vi "Main.vi"() -> ()   [LabVIEW 2020]
doc: "Example application with authentication."
uses:
  Type Definitions/States--enum.ctl
  Type Definitions/Loop Data--cluster.ctl
  <vilib>/gRPC/LabVIEW gRPC Library/Shared/grpcId.ctl
  <vilib>/sklein/WebView2/Webview2 Lib/WebView2 Control Object/WebView2 Control.lvclass
  <vilib>/Utility/miscctls.llb/LVPointTypeDef.ctl
  <vilib>/Utility/miscctls.llb/LVRectTypeDef.ctl
  grpc-auth_client/RPC Messages/auth_SubscribeLoginRequest.ctl
  grpc-auth_client/RPC Messages/auth_ValidateTokenRequest.ctl
  grpc-auth_client/RPC Messages/auth_RefreshTokenRequest.ctl
  grpc-auth_client/RPC Messages/auth_LogoutRequest.ctl
  e78014cf-5a62-4ef9-a1df-b3f489fcdea7.vi
  32d3baa6-2010-401a-92df-034dbfa07a08.vi
  <vilib>/Comparison/Equal/Equal Functor/Equal Functor.lvclass
  grpc-auth_client/grpc-auth_client.lvlib
  <vilib>/gRPC/LabVIEW gRPC Library/grpc-lvsupport-release.lvlib
  C:/Program Files (x86)/National Instruments/LabVIEW 2020/vi.lib/sklein/WebView2/Libs/Microsoft.Web.WebView2.WinForms.dll
  Program Files (x86)/National Instruments/LabVIEW 2020/vi.lib/sklein/WebView2/Libs/Microsoft.Web.WebView2.WinForms.dll
panel:
  in  "Tab Control":enum32{"Login", "Run"}(tab)
  in  "WebView2":refnum<k24>(container)
  in  "Extend":bool
  out "Access Expires At":string
  out "Current User":string
  out "In Operation":bool
  in  "operate":bool
  in  "debug":bool
  out "Debugging":bool
  in  "logout":bool
  # "Operation is only allowed\nfor members of group\n\"Operator\""
  # "Debugging is only allowed\nfor members of group\n\"Developers\""
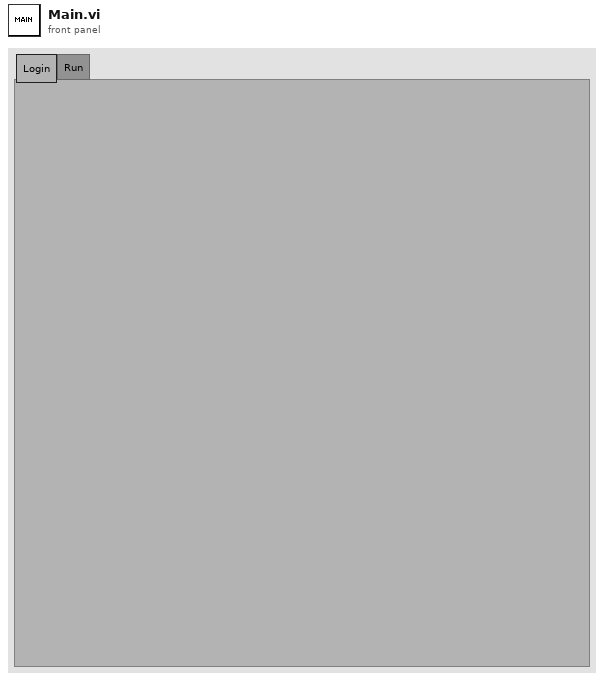
[diagram p1: front panel]
types:
  T1 = typedef "Loop Data--cluster.ctl" = cluster{"gRPC ID":T2, "Login Session ID":string, "Access Token":string, "Login Call ID":T2, "WebView2 Control":refnum<class "WebView2 Control.lvclass">}
  T2 = typedef "grpc-lvsupport-release.lvlib/grpcId.ctl" = u64
  T3 = typedef "States--enum.ctl" = enum16{"Init", "Login", "Idle", "Error", "Exit", "Begin SubscribeLogin", "End SubscribeLogin", "Logout"}
  T4 = typedef "LVRectTypeDef.ctl" = cluster{"Left":i16, "Top":i16, "Right":i16, "Bottom":i16}
  T5 = typedef "LVPointTypeDef.ctl" = cluster{"Horizontal":i16, "Vertical":i16}
  T6 = typedef "grpc-auth_client.lvlib/auth_SubscribeLoginRequest.ctl" = cluster{"session_id":string}
  T7 = typedef "grpc-auth_client.lvlib/auth_ValidateTokenRequest.ctl" = cluster{"access_token":string}
  T8 = typedef "grpc-auth_client.lvlib/auth_RefreshTokenRequest.ctl" = cluster{"access_token":string}
  T9 = typedef "grpc-auth_client.lvlib/auth_LogoutRequest.ctl" = cluster{"access_token":string}
  T10 = typedef "grpc-auth_client.lvlib/auth_StartLoginResponse.ctl" = cluster{"ok":bool, "error":string, "session_id":string, "login_url":string, "expires_at":i64}
  T11 = typedef "grpc-auth_client.lvlib/auth_ValidateTokenResponse.ctl" = cluster{"valid":bool, "error":string, "user_id":string, "groups":string[]}
  T12 = typedef "grpc-auth_client.lvlib/auth_SubscribeLoginResponse.ctl" = cluster{"ok":bool, "error":string, "status":T13, "access_token":string, "access_expires_at":i64, "username":string}
  T13 = typedef "grpc-auth_client.lvlib/auth_LoginStatus.ctl" = enum32{"LOGIN_STATUS_PENDING", "LOGIN_STATUS_READY", "LOGIN_STATUS_EXPIRED", "LOGIN_STATUS_USED", "LOGIN_STATUS_INVALID"}
  T14 = typedef "grpc-auth_client.lvlib/auth_RefreshTokenResponse.ctl" = cluster{"ok":bool, "error":string, "access_token":string, "access_expires_at":i64}
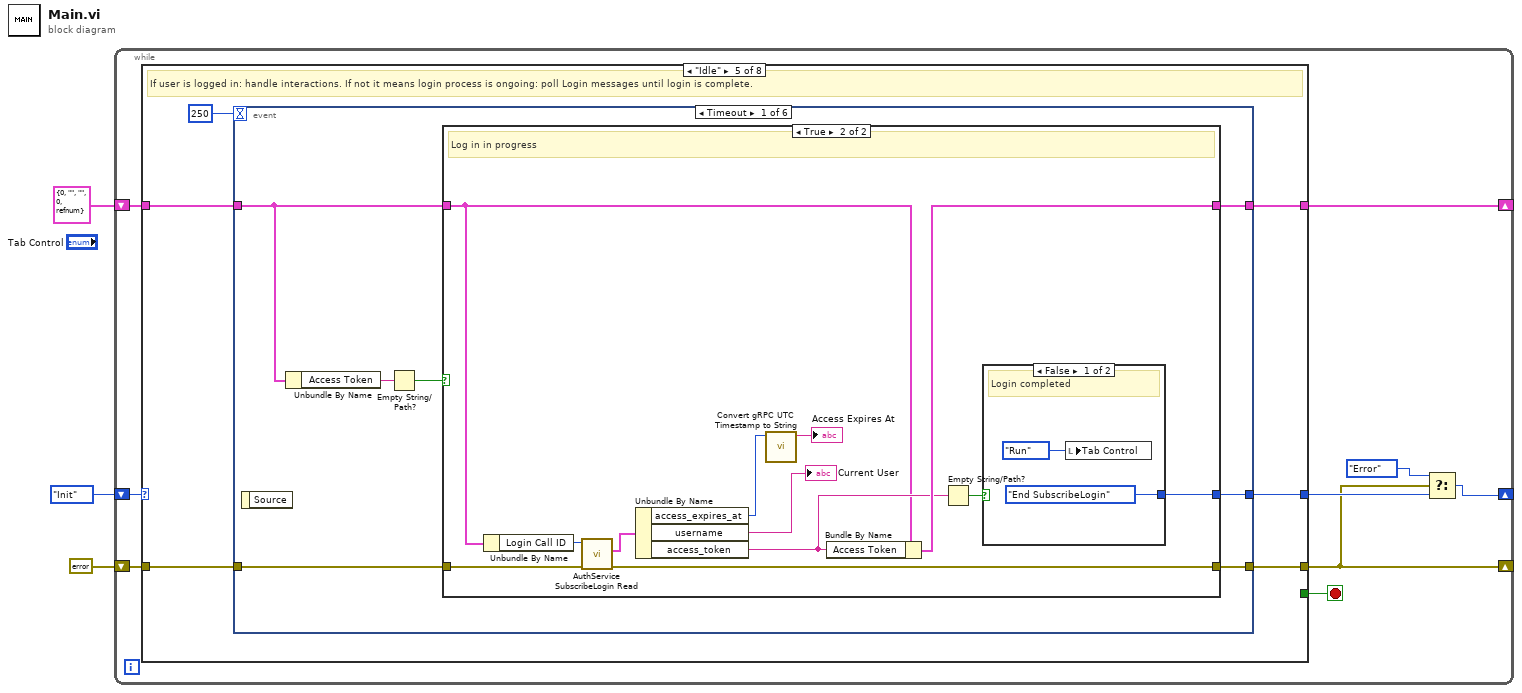
[diagram p0: block diagram]
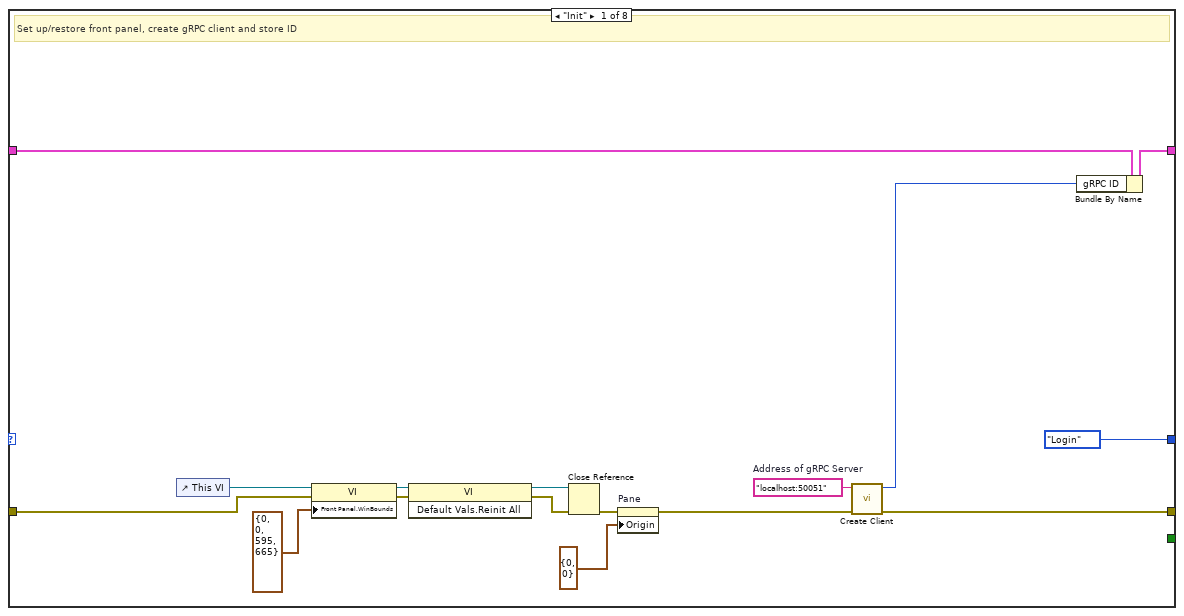
[diagram p2: hidden frame]
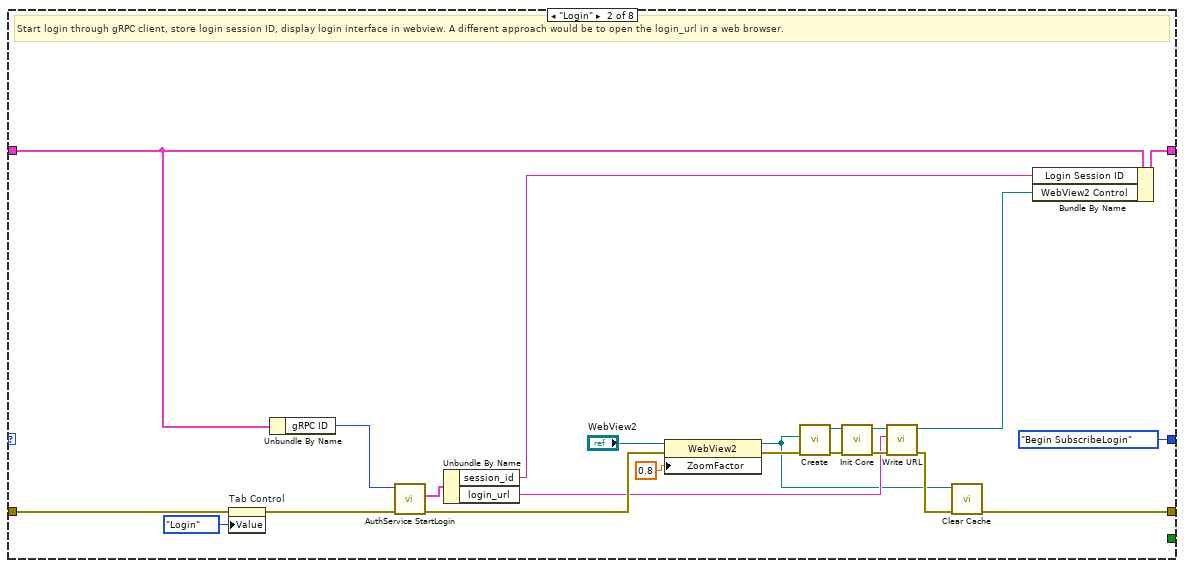
[diagram p3: hidden frame]
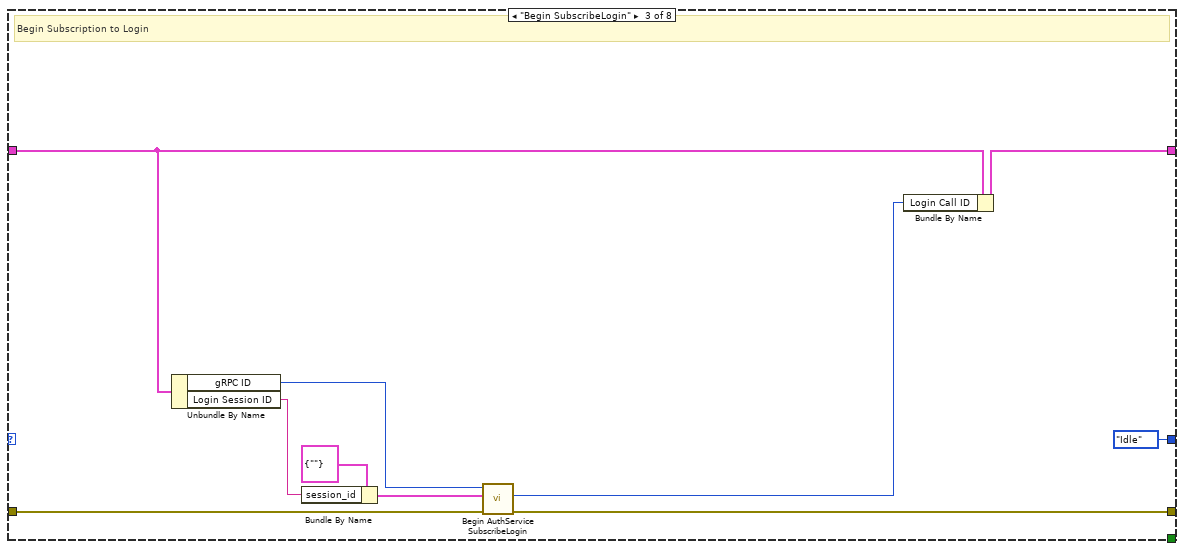
[diagram p4: hidden frame]
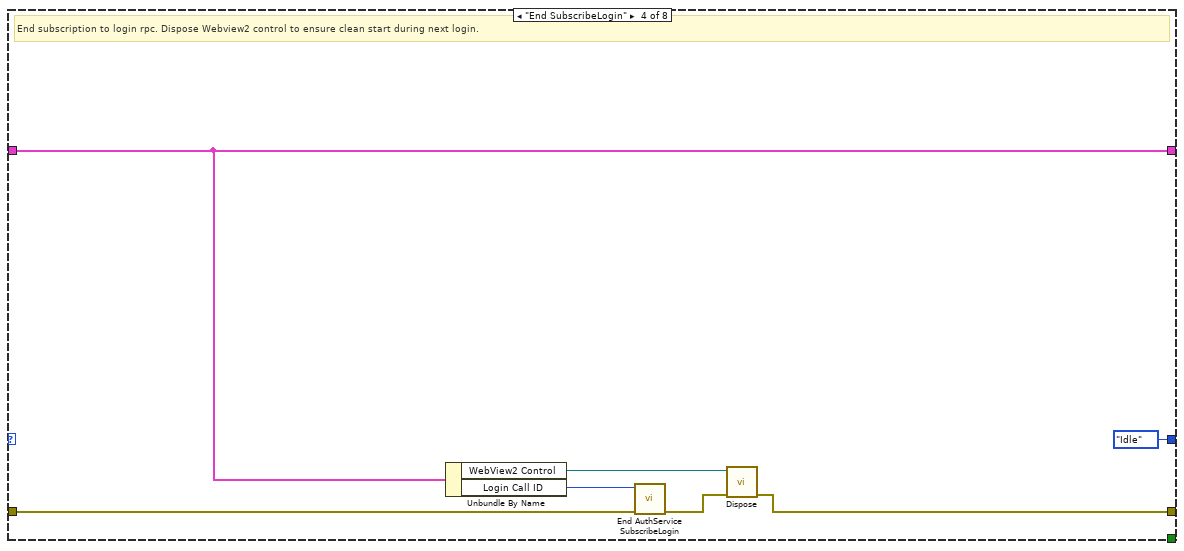
[diagram p5: hidden frame]
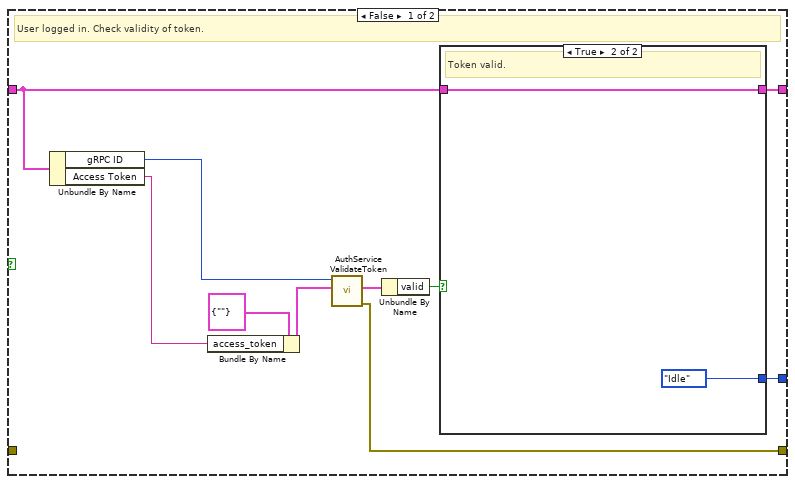
[diagram p6: hidden frame]
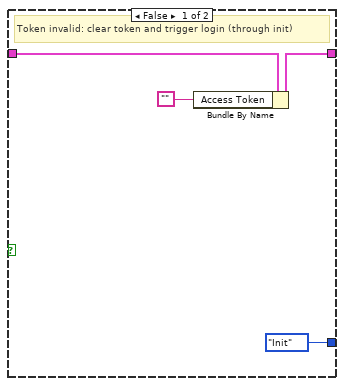
[diagram p7: hidden frame]
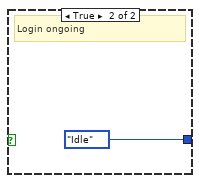
[diagram p8: hidden frame]
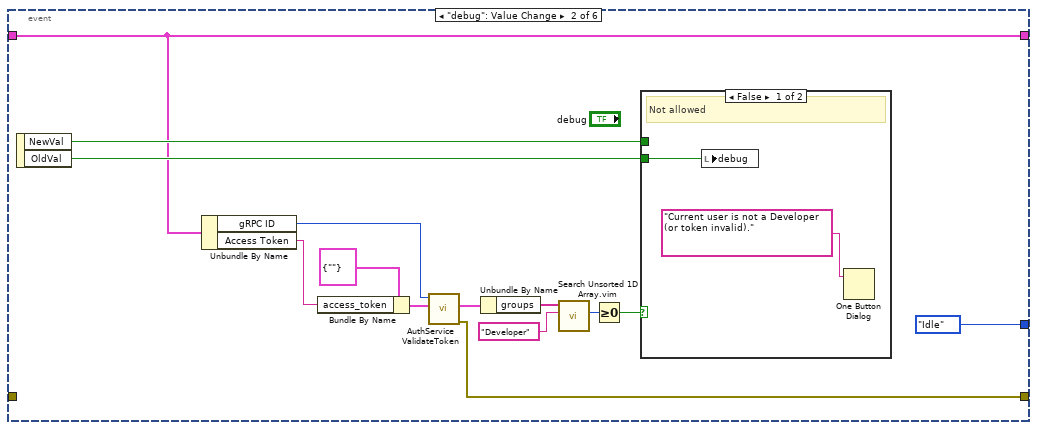
[diagram p9: hidden frame]
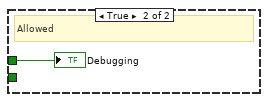
[diagram p10: hidden frame]
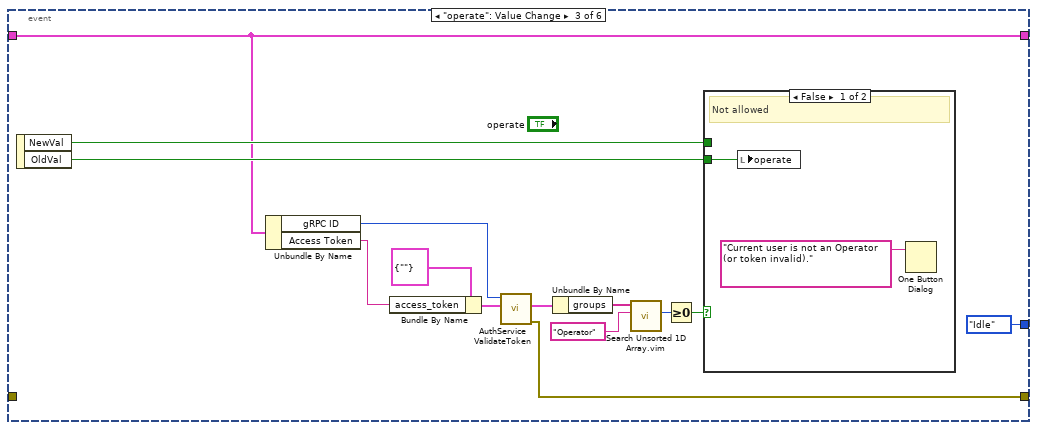
[diagram p11: hidden frame]
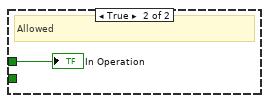
[diagram p12: hidden frame]
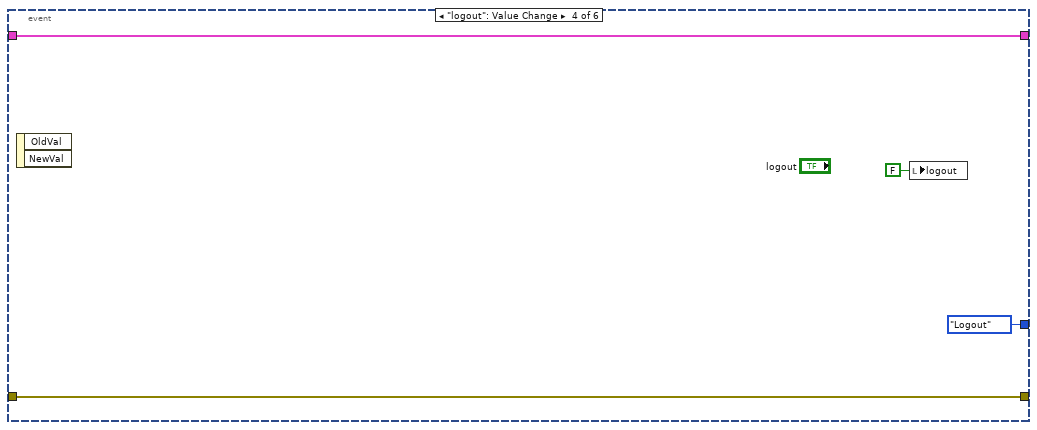
[diagram p13: hidden frame]
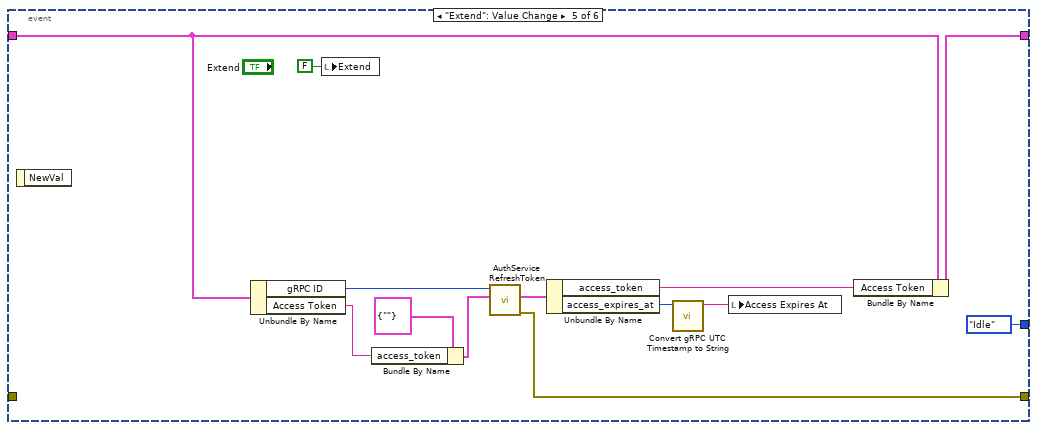
[diagram p14: hidden frame]
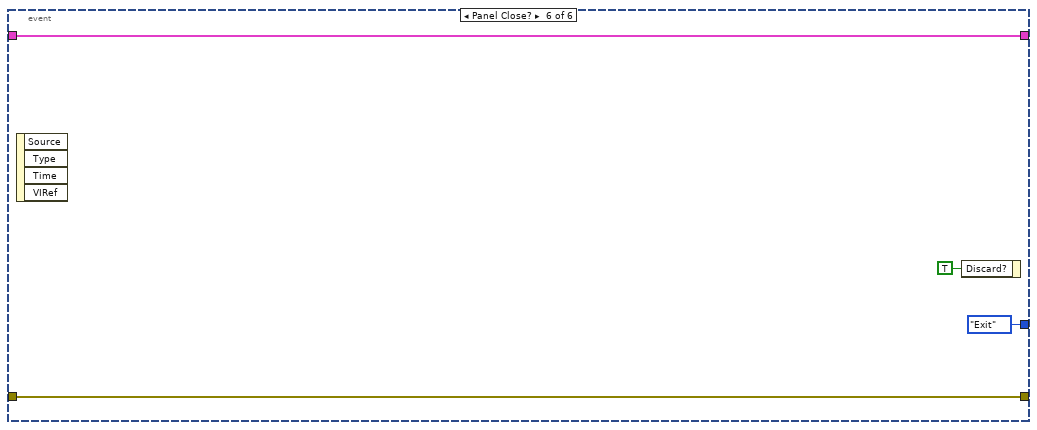
[diagram p15: hidden frame]
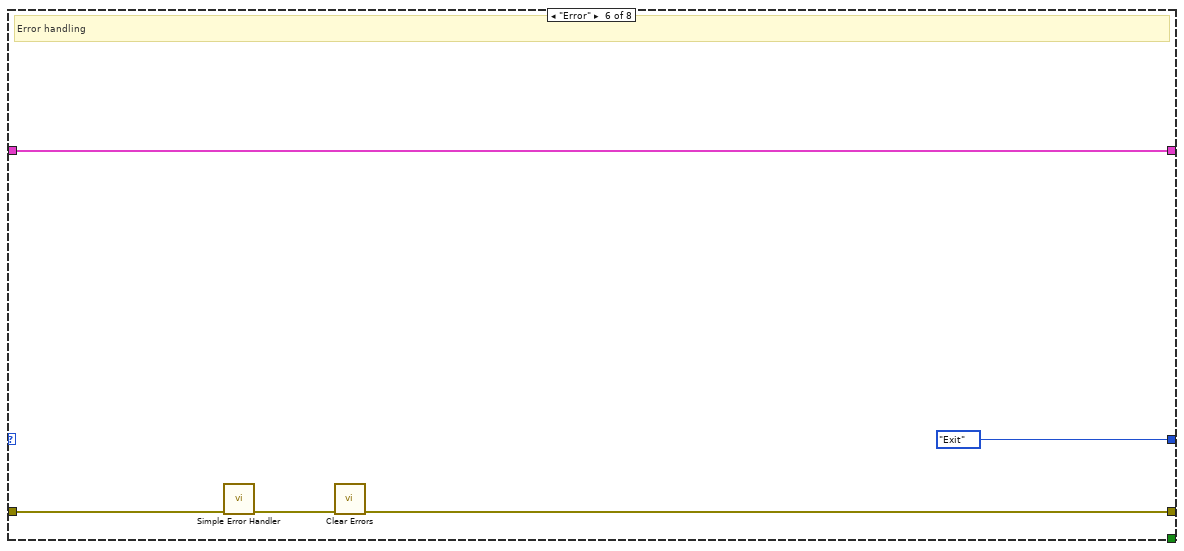
[diagram p16: hidden frame]
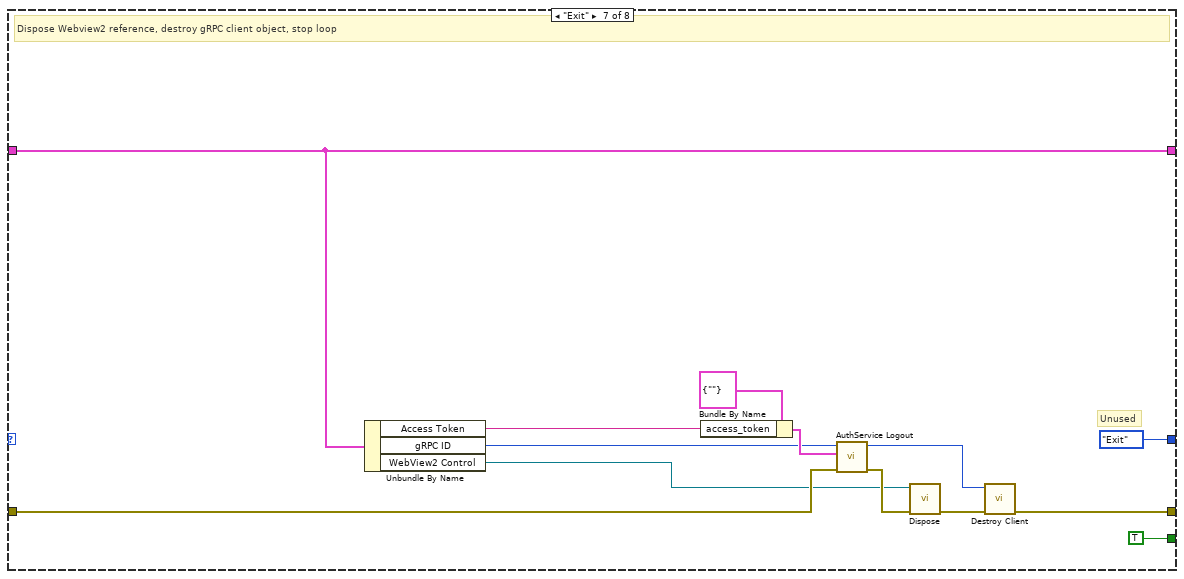
[diagram p17: hidden frame]
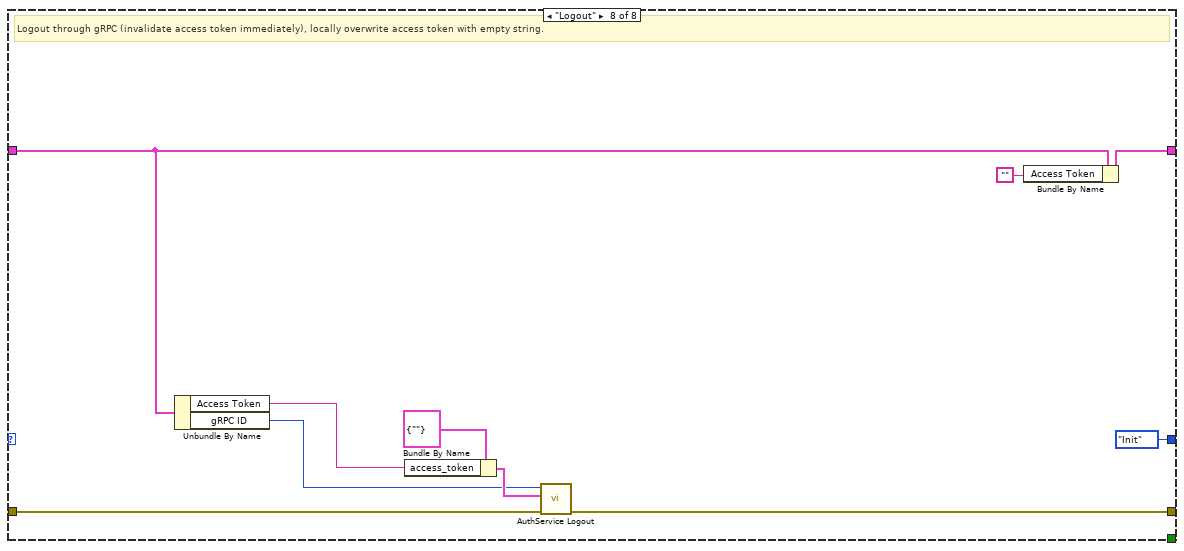
[diagram p18: hidden frame]
diagram:
  n1 = while {
    shift-right: [w9] -> _
    shift-left: States--enum."Init" -> [w12]
    shift-right: [w7] -> _
    shift-left: errorcluster {"status"=FALSE, "code"=0, "source"=""} ("error constant") -> [w11]
    shift-right: [w4] -> _
    shift-left: T1 {"gRPC ID"=0, "Login Session ID"="", "Access Token"="", "Login Call ID"=0, "WebView2 Control"=refnum} ("Loop Data") -> [w5]
    stop <- w6 stop-if-true
    n2 = case shown="\"Idle\"" w12 {
      tunnel: [w25 w42 w51 w62 w73 w169 w183 w185] -> w7
      tunnel: w11 -> [w19 w44 w60 w67 w71 w171 w175 w192]
      tunnel: [States--enum."Login" States--enum."Begin SubscribeLogin" States--enum."Idle" States--enum."Idle" w72 States--enum."Exit" States--enum."Exit" States--enum."Init"] -> w8
      tunnel: [_ _ _ _ _ _ TRUE _] -> w6
      tunnel: w5 -> [w22 w49 w55 w65 w70 w167 w181 w187]
      tunnel: [w23 w50 w54 w65 w69 w167 w181 w188] -> w4
      frame "Init" {
        w24 = "localhost:50051"  # Address of gRPC Server
        # "Set up/restore front panel, create gRPC client and store ID"
        n3 = control-ref of="This VI"() -> (w20:refnum<vi>)
        n4 = property on="Property Node" class="VI"(reference=w20, error in=w19, "Front Panel.WinBounds"=T4 {"Left"=0, "Top"=0, "Right"=595, "Bottom"=665} ("Front Panel Window:Window Bounds")) -> (reference out=w16:refnum<vi>, error out=w14:errorcluster)
        n5 = invoke on="Invoke Node" class="VI" method="Default Vals.Reinit All"(reference=w16, error in=w14) -> (reference out=w15:refnum<vi>, error out=w13:errorcluster)  [unwired: 1 in, 1 out]
        n6 = Close Reference(reference=w15, error in (no error)=w13) -> (error out=w18:errorcluster)
        n7 = property on="Pane" class="Pane"(error in=w18, "Origin"=T5 {"Horizontal"=0, "Vertical"=0}) -> (error out=w26:errorcluster)  [unwired: 1 in, 1 out]
        n8 = call "Create Client.vi"("error in"=w26, "address"=w24) -> ("error out"=w25:errorcluster, "gRPC ID Out"=w21:T2)  [unwired: 8 in]
        n9 = Bundle By Name(cluster=w22, "gRPC ID"=w21) -> (w23:T1)
      }
      frame "Login" {
        # "Start login through gRPC client, store login session ID, display login interface in webview. A different approach would be to open the login_url in a web browser."
        n10 = property on="Tab Control" class="TabCtl (strict)"(error in=w44, "Value"=enum32{"Login", "Run"}."Login" ("Tab Control")) -> (error out=w43:errorcluster)  [unwired: 1 in, 1 out]
        n11 = Unbundle By Name(w49) -> ("gRPC ID"=w48:T2)
        n12 = call "AuthService StartLogin.vi"("error in"=w43, "gRPC ID"=w48) -> ("error out"=w34:errorcluster, "Response Data"=w47:T10)  [unwired: 7 in, 1 out]
        n13 = Unbundle By Name(w47) -> ("session_id"=w46:string, "login_url"=w32:string)
        n14 = property on="Property Node" class="WebView2"(reference="WebView2", error in=w34, "ZoomFactor"=0.8) -> (reference out=w30:refnum<k24>, error out=w33:errorcluster)
        n15 = call <vilib>:"Create.vi"("error in (no error)"=w33, "WebView2 Control"=w30) -> ("error out"=w40:errorcluster, "WebView2 Control out"=w38:refnum<class "WebView2 Control.lvclass">)  [unwired: 8 in]
        n16 = call <vilib>:"Init Core.vi"("error in (no error)"=w40, "WebView2 Control in"=w38) -> ("error out"=w39:errorcluster, "WebView2 Control out"=w37:refnum<class "WebView2 Control.lvclass">)  [unwired: 8 in]
        n17 = call <vilib>:"Write URL.vi"("error in (no error)"=w39, "uri"=w32, "WebView2 Control in"=w37) -> ("error out"=w31:errorcluster, "WebView2 Control out"=w29:refnum<class "WebView2 Control.lvclass">)  [unwired: 7 in]
        n18 = call "Clear Cache.vi"("error in (no error)"=w31, ".NET Refnum in"=w30) -> ("error out"=w42:errorcluster)  [unwired: 9 in]
        n19 = Bundle By Name(cluster=w49, "Login Session ID"=w46, "WebView2 Control"=w29) -> (w50:T1)
      }
      frame "Begin SubscribeLogin" {
        # "Begin Subscription to Login"
        n20 = Unbundle By Name(w55) -> ("gRPC ID"=w59:T2, "Login Session ID"=w57:string)
        n21 = Bundle By Name(cluster=T6 {"session_id"=""} ("auth_SubscribeLoginRequest"), "session_id"=w57) -> (w56:T6)
        n22 = call "Begin AuthService SubscribeLogin.vi"("error in"=w60, "Request Data"=w56, "gRPC ID"=w59) -> ("error out"=w51:errorcluster, "Call Id Out"=w53:T2)  [unwired: 6 in, 1 out]
        n23 = Bundle By Name(cluster=w55, "Login Call ID"=w53) -> (w54:T1)
      }
      frame "End SubscribeLogin" {
        # "End subscription to login rpc. Dispose Webview2 control to ensure clean start during next login."
        n24 = Unbundle By Name(w65) -> ("WebView2 Control"=w61:refnum<class "WebView2 Control.lvclass">, "Login Call ID"=w64:T2)
        n25 = call "End AuthService SubscribeLogin.vi"("error in"=w67, "Call ID in"=w64) -> ("error out"=w63:errorcluster)  [unwired: 8 in, 1 out]
        n26 = call <vilib>:"Dispose.vi"("error in (no error)"=w63, "WebView2 Control in"=w61) -> ("error out"=w62:errorcluster)  [unwired: 9 in]
      }
      frame "Idle" {
        # "If user is logged in: handle interactions. If not it means login process is ongoing: poll Login messages until login is complete."
        n27 = event shown="[0] Timeout" {
          selector: _ -> [_ _ _ _ _ _]
          dyn-events: _ -> [_ _ _ _ _ _]
          timeout: 250 ("t") -> [_ _ _ _ _ _]
          tunnel: w70 -> [w76 w113 w130 w146 w153 w163]
          tunnel: [w80 w115 w132 w147 w150 w164] -> w73
          tunnel: [w77 States--enum."Idle" States--enum."Idle" States--enum."Logout" States--enum."Idle" States--enum."Exit"] -> w72
          tunnel: w71 -> [w79 _ _ w147 _ w164]
          tunnel: [w78 w113 w130 w146 w154 w163] -> w69
          event Timeout {
            n28 = event-data() -> ()  [unwired: 1 in, 1 out]
            n29 = Unbundle By Name(w76) -> ("Access Token"=w75:string)
            n30 = Empty String/Path?(string/path=w75) -> (empty?=w74:bool)
            n31 = case shown="True" w74 {
              tunnel: [w83 w108] -> w80
              tunnel: w79 -> [_ w107]
              tunnel: [w82 w104] -> w78
              tunnel: [w84 w100] -> w77
              tunnel: w76 -> [w81 w97]
              frame False {
                # "User logged in. Check validity of token."
                n32 = Unbundle By Name(w81) -> ("gRPC ID"=w90:T2, "Access Token"=w88:string)
                n33 = Bundle By Name(cluster=T7 {"access_token"=""} ("auth_ValidateTokenRequest"), "access_token"=w88) -> (w87:T7)
                n34 = call "AuthService ValidateToken.vi"("Request Data"=w87, "gRPC ID"=w90) -> ("error out"=w83:errorcluster, "Response Data"=w86:T11)  [unwired: 7 in, 1 out]
                n35 = Unbundle By Name(w86) -> ("valid"=w85:bool)
                n36 = case shown="True" w85 {
                  tunnel: [States--enum."Init" ("f") States--enum."Idle" ("f")] -> w84
                  tunnel: [w91 w95] -> w82
                  tunnel: w81 -> [w93 w95]
                  frame False {
                    # "Token invalid: clear token and trigger login (through init)"
                    n37 = Bundle By Name(cluster=w93, "Access Token"="" ("Empty String Constant")) -> (w91:T1)
                  }
                  frame True {
                    # "Token valid."
                  }
                }
              }
              frame True {
                # "Log in in progress"
                n38 = Unbundle By Name(w97) -> ("Login Call ID"=w106:T2)
                n39 = call "AuthService SubscribeLogin Read.vi"("error in"=w107, "Call ID in"=w106) -> ("error out"=w108:errorcluster, "Response Data"=w105:T12)  [unwired: 6 in, 2 out]
                n40 = Unbundle By Name(w105) -> ("access_expires_at"=w99:i64, "username"=→"Current User":string, "access_token"=w103:string)
                n41 = call "Convert gRPC UTC Timestamp to String.vi"("access_expires_at"=w99) -> ("date/time string"=→"Access Expires At":string)  [unwired: 10 in]
                n42 = Bundle By Name(cluster=w97, "Access Token"=w103) -> (w104:T1)
                n43 = Empty String/Path?(string/path=w103) -> (empty?=w101:bool)
                n44 = case shown="False" w101 {
                  tunnel: [States--enum."End SubscribeLogin" ("f") States--enum."Idle" ("f")] -> w100
                  frame False {
                    # "Login completed"
                    n45 = local write "Tab Control"(enum32{"Login", "Run"}."Run" ("Tab Control")) -> ()
                  }
                  frame True {
                    # "Login ongoing"
                  }
                }
              }
            }
          }
          event "debug": Value Change {
            n46 = event-data() -> ("NewVal"=w117:bool, "OldVal"=w114:bool)  [unwired: 1 in]
            n47 = Unbundle By Name(w113) -> ("gRPC ID"=w124:T2, "Access Token"=w112:string)
            n48 = Bundle By Name(cluster=T7 {"access_token"=""} ("auth_ValidateTokenRequest"), "access_token"=w112) -> (w125:T7)
            n49 = call "AuthService ValidateToken.vi"("Request Data"=w125, "gRPC ID"=w124) -> ("error out"=w115:errorcluster, "Response Data"=w123:T11)  [unwired: 7 in, 1 out]
            n50 = Unbundle By Name(w123) -> ("groups"=w122:string[])
            n51 = call "Search Unsorted 1D Array.vim"("element"="Developer", "unsorted 1D array"=w122) -> ("index of element"=w121:i32)  [unwired: 9 in]
            n52 = Greater Or Equal To 0?(x=w121) -> (x >= 0?=w118:bool)
            n53 = case shown="False" w118 {
              tunnel: w117 -> [_ w128]
              tunnel: w114 -> [w127 _]
              frame False {
                # "Not allowed"
                n54 = local write "debug"(w127) -> ()
                n55 = One Button Dialog(message="Current user is not a Developer (or token invalid)." ("format string")) -> ()  [unwired: 1 in, 1 out]
              }
              frame True {
                # "Allowed"
                "Debugging" <- w128
              }
            }
          }
          event "operate": Value Change {
            n56 = event-data() -> ("NewVal"=w134:bool, "OldVal"=w131:bool)  [unwired: 1 in]
            n57 = Unbundle By Name(w130) -> ("gRPC ID"=w141:T2, "Access Token"=w129:string)
            n58 = Bundle By Name(cluster=T7 {"access_token"=""} ("auth_ValidateTokenRequest"), "access_token"=w129) -> (w142:T7)
            n59 = call "AuthService ValidateToken.vi"("Request Data"=w142, "gRPC ID"=w141) -> ("error out"=w132:errorcluster, "Response Data"=w140:T11)  [unwired: 7 in, 1 out]
            n60 = Unbundle By Name(w140) -> ("groups"=w139:string[])
            n61 = call "Search Unsorted 1D Array.vim"("element"="Operator", "unsorted 1D array"=w139) -> ("index of element"=w138:i32)  [unwired: 9 in]
            n62 = Greater Or Equal To 0?(x=w138) -> (x >= 0?=w135:bool)
            n63 = case shown="False" w135 {
              tunnel: w134 -> [_ w145]
              tunnel: w131 -> [w143 _]
              frame False {
                # "Not allowed"
                n64 = local write "operate"(w143) -> ()
                n65 = One Button Dialog(message="Current user is not an Operator (or token invalid)." ("format string")) -> ()  [unwired: 1 in, 1 out]
              }
              frame True {
                # "Allowed"
                "In Operation" <- w145
              }
            }
          }
          event "logout": Value Change {
            n66 = event-data() -> ()  [unwired: 1 in, 2 out]
            n67 = local write "logout"(FALSE ("logout")) -> ()
          }
          event "Extend": Value Change {
            n68 = event-data() -> ()  [unwired: 1 in, 1 out]
            n69 = Unbundle By Name(w153) -> ("gRPC ID"=w161:T2, "Access Token"=w159:string)
            n70 = local write "Extend"(FALSE ("Extend")) -> ()
            n71 = Bundle By Name(cluster=T8 {"access_token"=""} ("auth_RefreshTokenRequest"), "access_token"=w159) -> (w158:T8)
            n72 = call "AuthService RefreshToken.vi"("Request Data"=w158, "gRPC ID"=w161) -> ("error out"=w150:errorcluster, "Response Data"=w157:T14)  [unwired: 7 in, 1 out]
            n73 = Unbundle By Name(w157) -> ("access_token"=w152:string, "access_expires_at"=w156:i64)
            n74 = call "Convert gRPC UTC Timestamp to String.vi"("access_expires_at"=w156) -> ("date/time string"=w155:string)  [unwired: 10 in]
            n75 = local write "Access Expires At"(w155) -> ()
            n76 = Bundle By Name(cluster=w153, "Access Token"=w152) -> (w154:T1)
          }
          event Panel Close? {
            n77 = event-data() -> ()  [unwired: 1 in, 4 out]
            n78 = event-data ("Event Filter Node")("Discard?"=TRUE) -> ()  [unwired: 1 in, 1 out]
          }
        }
      }
      frame "Error" {
        # "Error handling"
        n79 = call <vilib>:"Simple Error Handler.vi"("error in (no error)"=w171) -> ("error out"=w170:errorcluster)  [unwired: 4 in, 4 out]
        n80 = call <vilib>:"Clear Errors.vi"("error in (no error)"=w170) -> ("error out"=w169:errorcluster)  [unwired: 5 in, 1 out]
      }
      frame "Exit" {
        # "Unused"
        # "Dispose Webview2 reference, destroy gRPC client object, stop loop"
        n81 = Unbundle By Name(w181) -> ("Access Token"=w178:string, "gRPC ID"=w176:T2, "WebView2 Control"=w172:refnum<class "WebView2 Control.lvclass">)
        n82 = Bundle By Name(cluster=T9 {"access_token"=""} ("auth_LogoutRequest"), "access_token"=w178) -> (w179:T9)
        n83 = call "AuthService Logout.vi"("error in"=w175, "Request Data"=w179, "gRPC ID"=w176) -> ("error out"=w174:errorcluster, "gRPC ID out"=w177:T2)  [unwired: 6 in, 1 out]
        n84 = call <vilib>:"Dispose.vi"("error in (no error)"=w174, "WebView2 Control in"=w172) -> ("error out"=w173:errorcluster)  [unwired: 9 in]
        n85 = call "Destroy Client.vi"("error in"=w173, "gRPC ID"=w177) -> ("error out"=w183:errorcluster)  [unwired: 9 in]
      }
      frame "Logout" {
        # "Logout through gRPC (invalidate access token immediately), locally overwrite access token with empty string."
        n86 = Unbundle By Name(w187) -> ("Access Token"=w190:string, "gRPC ID"=w191:T2)
        n87 = Bundle By Name(cluster=T9 {"access_token"=""} ("auth_LogoutRequest"), "access_token"=w190) -> (w193:T9)
        n88 = call "AuthService Logout.vi"("error in"=w192, "Request Data"=w193, "gRPC ID"=w191) -> ("error out"=w185:errorcluster)  [unwired: 6 in, 2 out]
        n89 = Bundle By Name(cluster=w187, "Access Token"="" ("Empty String Constant")) -> (w188:T1)
      }
    }
    n90 = Select(t=States--enum."Error", s=w7, f=w8) -> (s? t:f=w9:T3)
  }
